vi "Error Test Number Of Bits.vi"(2 "direction":T1, 5 "number of bits":i32, 9 "start bit":i32, 11 "error in":errorcluster, 12 "error text in":string) -> (15 "error out":errorcluster)   [LabVIEW 2023]
uses:
  Direction.ctl
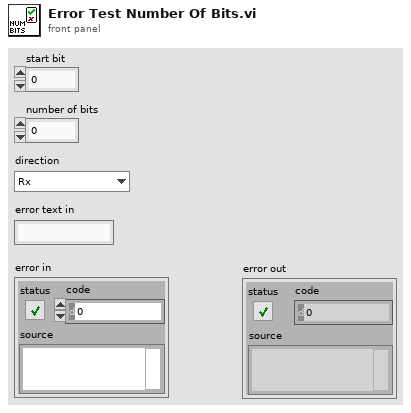
[diagram p1: front panel]
types:
  T1 = typedef "Direction.ctl" = enum16{"Rx", "Tx"}
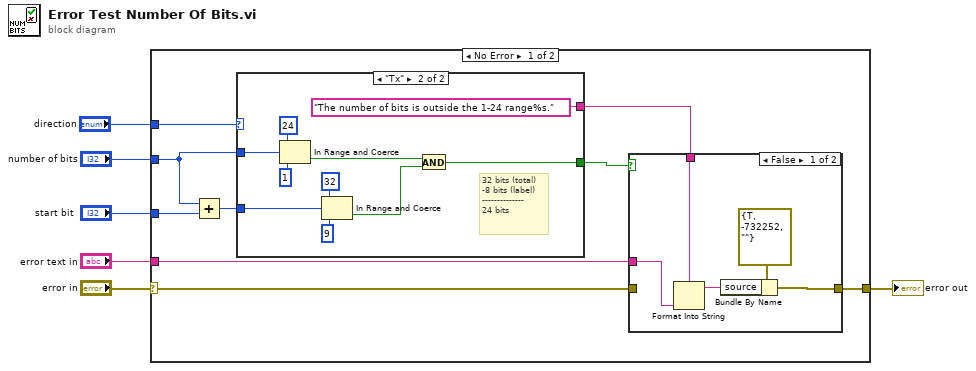
[diagram p0: block diagram]
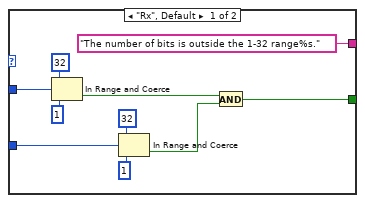
[diagram p3: hidden frame]
diagram:
  n1 = case shown="No Error" "error in" {
    selector: "error in" -> [w15 w42]
    tunnel: [w14 w42] -> w5
    tunnel: "number of bits" -> [w8 _]
    tunnel: "error text in" -> [w12 _]
    tunnel: "direction" -> [w11 _]
    tunnel: "start bit" -> [w9 _]
    frame No Error {
      n2 = Add(x=w8, y=w9) -> (x+y=w7:i32)
      n3 = case shown="\"Tx\"" w11 {
        tunnel: w8 -> [w31 w41]
        tunnel: [w22 w32] -> w13
        tunnel: ["The number of bits is outside the 1-32 range%s." ("source") "The number of bits is outside the 1-24 range%s." ("source")] -> w10
        tunnel: w7 -> [w25 w34]
        frame "Rx", Default {
          n4 = In Range and Coerce(upper limit=32 ("lower limit"), x=w31, lower limit=1) -> (In Range?=w24:bool)  [unwired: 1 out]
          n5 = In Range and Coerce(upper limit=32 ("lower limit"), x=w25, lower limit=1) -> (In Range?=w23:bool)  [unwired: 1 out]
          n6 = And(x=w24, y=w23) -> (x .and. y?=w22:bool)
        }
        frame "Tx" {
          # "32 bits (total)\n-8 bits (label)\n--------------\n24 bits"
          n7 = In Range and Coerce(upper limit=24 ("lower limit"), x=w41, lower limit=1) -> (In Range?=w33:bool)  [unwired: 1 out]
          n8 = In Range and Coerce(upper limit=32 ("lower limit"), x=w34, lower limit=9) -> (In Range?=w35:bool)  [unwired: 1 out]
          n9 = And(x=w33, y=w35) -> (x .and. y?=w32:bool)
        }
      }
      n10 = case shown="False" w13 {
        tunnel: w15 -> [_ w21]
        tunnel: [w20 w21] -> w14
        tunnel: w12 -> [w19 _]
        tunnel: w10 -> [w17 _]
        frame False {
          n11 = Format Into String(format string=w17, w19) -> (resulting string=w18:string)  [unwired: 2 in, 1 out]
          n12 = Bundle By Name(cluster=errorcluster {"status"=TRUE, "code"=-732252, "source"=""} ("error constant"), "source"=w18) -> (w20:errorcluster)
        }
        frame True {
        }
      }
    }
    frame Error {
    }
  }
  "error out" <- w5
